vi "Reset Results.vi"(8 "error in":errorcluster, 11 "Sequence Executor in":refnum<class "Sequence Executor.lvclass">) -> (0 "error out":errorcluster, 3 "Sequence Executor out":refnum<class "Sequence Executor.lvclass">)   [LabVIEW 2026, in "Sequence Executor.lvclass"]
doc: "Helper. Rebuilds Results from Sequence.steps: one Step Result per step with result NOT RUN, empty reason and zero numbers."
uses:
  Sequence Executor.lvclass
  Sequence Executor.lvclass/Sequence Executor.ctl
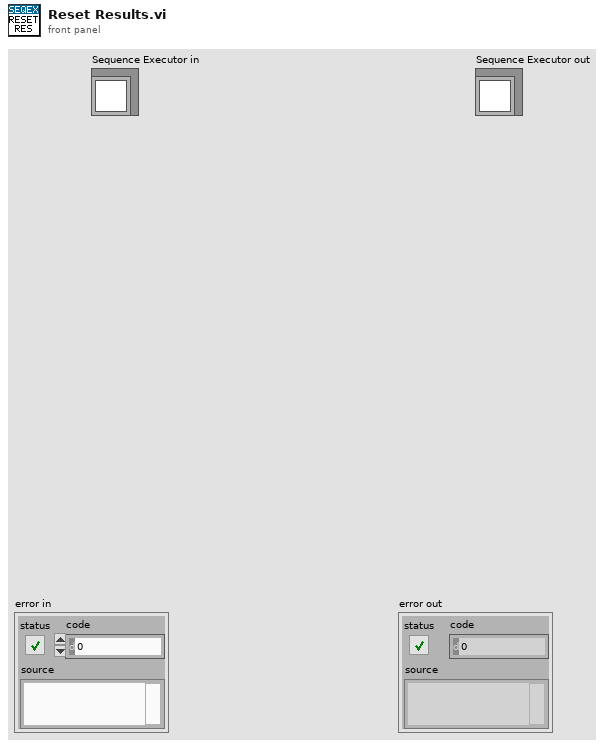
[diagram p1: front panel]
types:
  T1 = typedef "Sequence File.ctl" = cluster{"sequence_id":string, "description":string, "total_steps":i32, "steps":T2[]}
  T2 = typedef "Step Config.ctl" = cluster{"step_no":i32, "step_name":string, "command_type":string, "pressure_sp_bar":dbl, "flow_sp_lpm":dbl, "displacement_sp_mm":dbl, "monitored_io":string, "tolerance_bar":dbl, "dwell_time_ms":i32, "timeout_ms":i32, "expected_result":string}
  T3 = cluster{"step_no":i32, "step_name":string, "result":string, "reason":string, "measured":dbl, "target":dbl, "duration_ms":dbl}
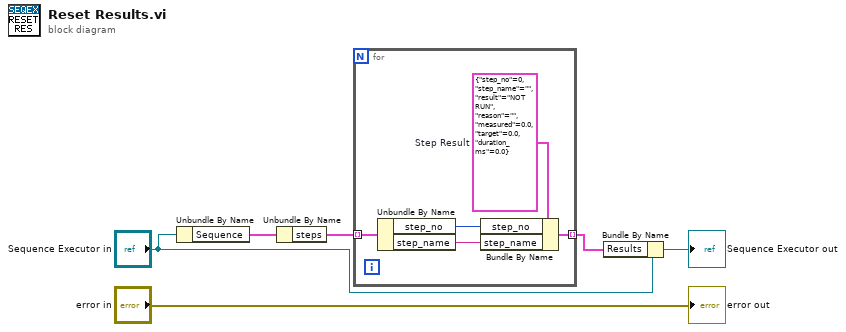
[diagram p0: block diagram]
diagram:
  n1 = Unbundle By Name("Sequence Executor in") -> ("Sequence"=w6:T1)
  n2 = Unbundle By Name(w6) -> ("steps"=w5:T2[])
  n3 = for {
    tunnel: w5 -> [w11] mode=indexing
    tunnel: [w7] -> w4 mode=indexing
    w8 = T3 {"step_no"=0, "step_name"="", "result"="NOT RUN", "reason"="", "measured"=0.0, "target"=0.0, "duration_ms"=0.0}  # Step Result
    n4 = Unbundle By Name(w11) -> ("step_no"=w10:i32, "step_name"=w9:string)
    n5 = Bundle By Name(cluster=w8, "step_no"=w10, "step_name"=w9) -> (w7:T3)
  }
  n6 = Bundle By Name(cluster="Sequence Executor in", "Results"=w4) -> (→"Sequence Executor out":refnum<class "Sequence Executor.lvclass">)
  "error out" <- "error in"
